vi "Get Tx Hardware Channel Data.vi"(8 "error in":errorcluster, 11 "custom device ref in":T7 format="%.0x") -> (0 "error out":errorcluster, 1 "Tx hardware channel data":T1[](array[typedef]) {"labels settings for RT"."Label Timestamp Channel Data Reference" format="%.0x"; "labels settings for RT"."Word Initial Raw Value" format="%032.0f"; "labels settings for RT"."Label Disable/Trigger Channel Reference" format="%.0x"; "labels settings for RT"."parameter driver data"."Tx parameter refs" format="%.0x"; "labels settings for RT"."SDI" format="%02b"; "labels settings for RT"."label" format="%.0o"}, 3 "custom device ref out":T7 format="%.0x")   [LabVIEW 2020]
uses:
  <vilib>/NI VeriStand/Custom Device API/Custom Device Item Ref.ctl
  RT Hardware Channel Settings.ctl
  RT Label Settings.ctl
  Label.ctl
  RT Parameters.ctl
  Parameter Definition.ctl
  <vilib>/NI/NI VeriStand Encoding and Decoding/Encoding.ctl
  Transfer Type.ctl
  <vilib>/NI VeriStand/Custom Device API/Data Reference.ctl
  Transfer Speed.ctl
  Scripting/AIM/AIM ARINC 429 Scripting.lvlib
  <vilib>/NI VeriStand/Custom Device API/Custom Device API.lvlib
  <vilib>/NI/NI VeriStand Encoding and Decoding/Encoding and Decoding.lvlib
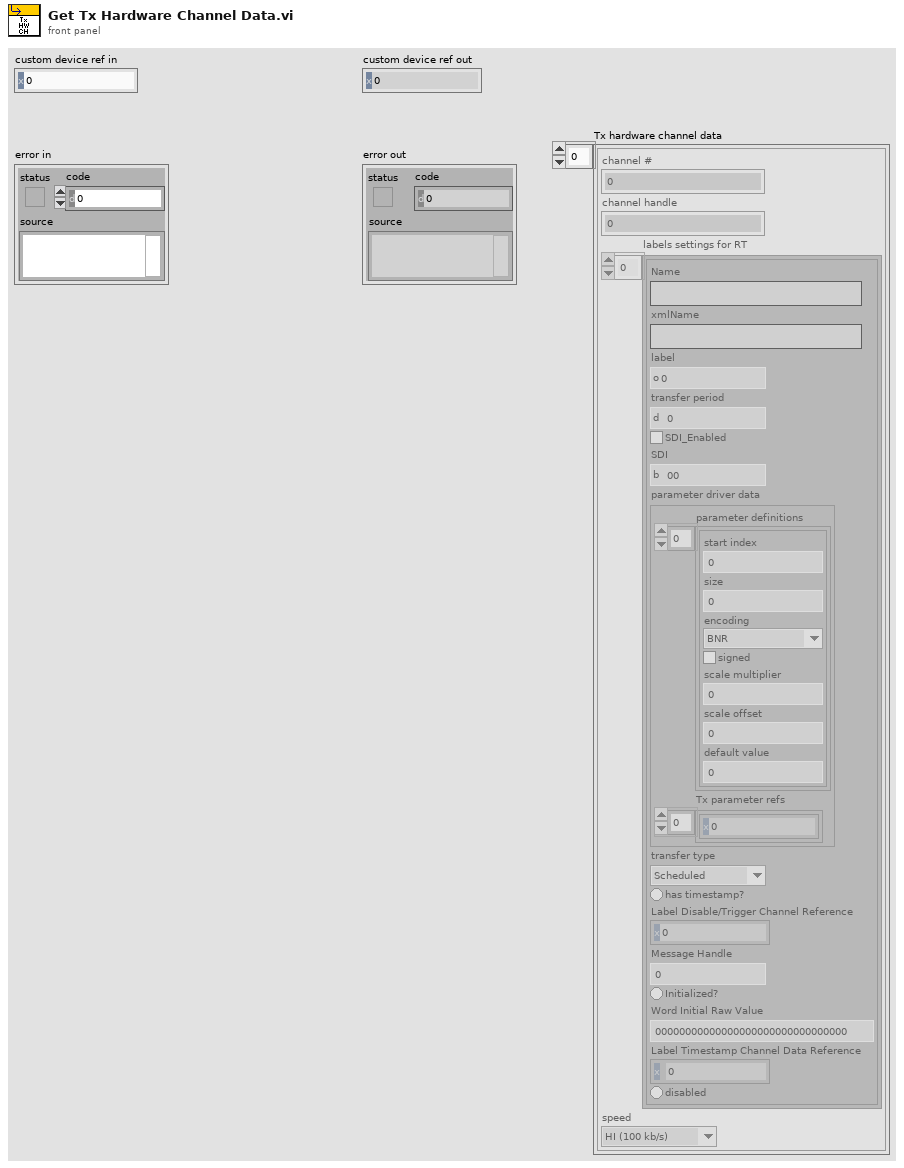
[diagram p1: front panel]
types:
  T1 = typedef "RT Hardware Channel Settings.ctl" = cluster{"channel #":u16, "channel handle":u64, "labels settings for RT":T2[], "speed":T10}
  T2 = typedef "RT Label Settings.ctl" = cluster{"Name":string, "xmlName":string, "label":T3, "transfer period":u32, "SDI_Enabled":bool, "SDI":u8, "parameter driver data":T4, "transfer type":T8, "has timestamp?":bool, "Label Disable/Trigger Channel Reference":T7, "Message Handle":u64, "Initialized?":bool, "Word Initial Raw Value":u32, "Label Timestamp Channel Data Reference":T9, "disabled":bool}
  T3 = typedef "Label.ctl" = u8
  T4 = typedef "RT Parameters.ctl" = cluster{"parameter definitions":T5[], "Tx parameter refs":T7[]}
  T5 = typedef "Parameter Definition.ctl" = cluster{"start index":i32, "size":i32, "encoding":T6, "signed":bool, "scale multiplier":dbl, "scale offset":dbl, "default value":dbl}
  T6 = typedef "Encoding and Decoding.lvlib/Encoding.ctl" = enum16{"BNR", "BCD", "Discrete"}
  T7 = typedef "Custom Device API.lvlib/Custom Device Item Ref.ctl" = u64
  T8 = typedef "Transfer Type.ctl" = enum16{"Scheduled", "Acyclic", "Block", "Strobe"}
  T9 = typedef "Custom Device API.lvlib/Data Reference.ctl" = i32
  T10 = typedef "Transfer Speed.ctl" = enum16{"LO (12.5 kb/s)", "HI (100 kb/s)"}
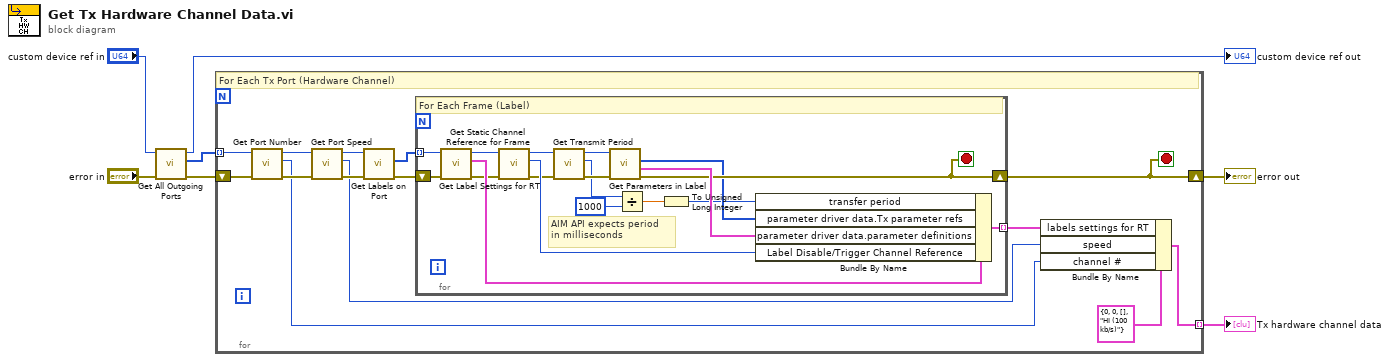
[diagram p0: block diagram]
diagram:
  n1 = call "Get All Outgoing Ports.vi"("error in"="error in", "custom device ref"="custom device ref in") -> ("error out"=w5:errorcluster, "outgoing ports"=w4:T7[], "custom device ref out"=→"custom device ref out":T7)  [unwired: 7 in]
  n2 = for {
    shift-right: [w21] -> w1
    shift-left: w5 -> [w16]
    tunnel: w4 -> [w17] mode=indexing
    tunnel: [w20] -> w6 mode=indexing
    stop <- w21 stop-if-true
    # "For Each Tx Port (Hardware Channel)"
    n3 = call "Get Port Number.vi"("error in"=w16, "port ref"=w17) -> ("error out"=w13:errorcluster, "port number"=w9:u16, "port ref out"=w12:T7)  [unwired: 6 in, 1 out]
    n4 = call "Get Port Speed.vi"("error in"=w13, "port ref"=w12) -> ("error out"=w10:errorcluster, "speed"=w8:T10, "port ref out"=w11:T7)  [unwired: 7 in]
    n5 = call "Get Labels on Port.vi"("error in"=w10, "port ref"=w11) -> ("error out"=w14:errorcluster, "labels"=w15:T7[])  [unwired: 6 in, 2 out]
    n6 = for {
      tunnel: w15 -> [w26] mode=indexing
      shift-right: [w33] -> w21
      shift-left: w14 -> [w39]
      tunnel: [w36] -> w19 mode=indexing
      stop <- w33 stop-if-true
      # "AIM API expects period\nin milliseconds"
      # "For Each Frame (Label)"
      n7 = call "Get Label Settings for RT.vi"("error in"=w39, "label ref in"=w26) -> ("error out"=w35:errorcluster, "label settings for RT"=w38:T2, "label ref out"=w27:T7)  [unwired: 7 in]
      n8 = call "Get Static Channel Reference for Frame.vi"("error in"=w35, "label ref"=w27) -> ("error out"=w31:errorcluster, "channel specification ref"=w34:T7, "label ref out"=w28:T7)  [unwired: 6 in, 1 out]
      n9 = call "Get Transmit Period.vi"("error in"=w31, "label ref"=w28) -> ("error out"=w30:errorcluster, "transmit period (us)"=w25:u32, "label ref out"=w29:T7)  [unwired: 7 in]
      n10 = call "Get Parameters in Label.vi"("error in"=w30, "label ref"=w29) -> ("error out"=w33:errorcluster, "parameter definitions"=w37:T5[], "parameters"=w32:T7[])  [unwired: 6 in, 1 out]
      n11 = Divide(x=w25, y=u32 1000) -> (x/y=w23:dbl)
      n12 = To Unsigned Long Integer(number=w23) -> (unsigned 32bit integer=w22:u32)
      n13 = Bundle By Name(cluster=w38, "transfer period"=w22, "parameter driver data.Tx parameter refs"=w32, "parameter driver data.parameter definitions"=w37, "Label Disable/Trigger Channel Reference"=w34) -> (w36:T2)
    }
    n14 = Bundle By Name(cluster=T1 {"channel #"=0, "channel handle"=0, "labels settings for RT"=[], "speed"=enum."HI (100 kb/s)"} ("RT hardware channel"), "labels settings for RT"=w19, "speed"=w8, "channel #"=w9) -> (w20:T1)
  }
  "error out" <- w1
  "Tx hardware channel data" <- w6
